vi "csb frames to pcap.vi"(0 "n_frames":i32, 1 "t_dev":dbl[](array[numeric]), 2 "id":u32[](array[numeric]), 3 "flags":u16[](array[numeric]), 4 "data_len":u8[](array[numeric]), 5 "data":u8[](array[numeric]), 6 "tai_minus_utc_s":i32, 7 "error in (no error)":errorcluster, 8 "options":i32, 9 "out":u8[](array[numeric])=array[4097 elements], 10 "out_cap":i32) -> (19 "out out":u8[](array[numeric]), 20 "n_packets":i32, 21 "n_skipped":i32, 22 "function return":i32, 27 "error out":errorcluster)   [LabVIEW 2021, in "CANsub_Codec.lvlib"]
doc: "int32_t csb_frames_to_pcap(int32_t n_frames, const double *t_dev, const uint32_t *id,\n const uint16_t *flags, const uint8_t *data_len, const uint8_t *data,\n int32_t tai_minus_utc_s, int32_t options,\n uint8_t *out, int32_t out_cap, int32_t *n_packets, int32_t *n_skipped);"
uses:
  CANsub_Codec.lvlib
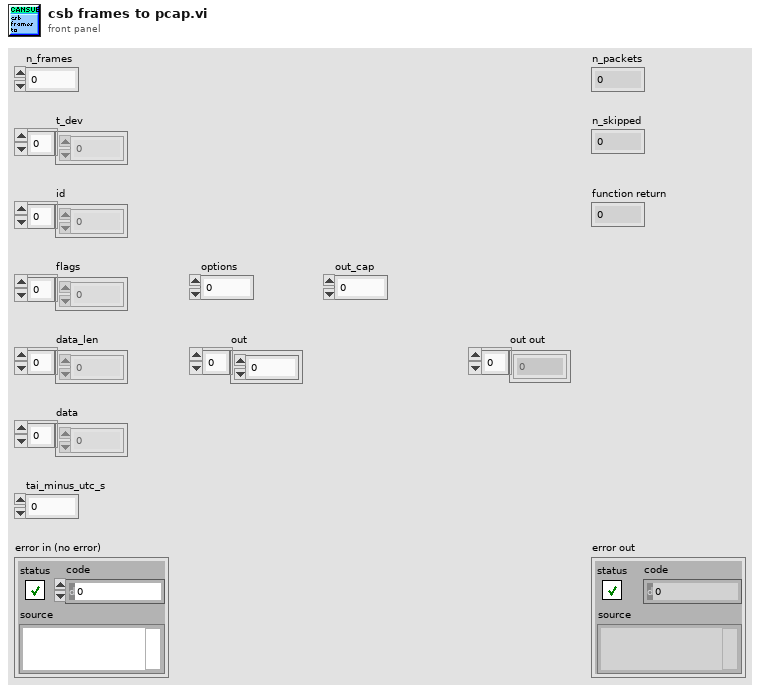
[diagram p1: front panel]
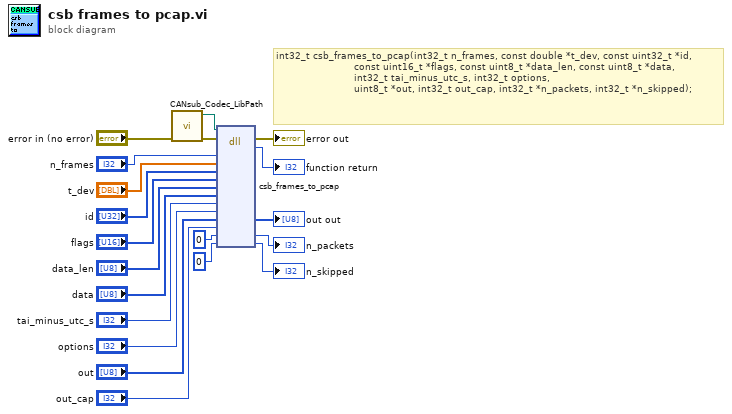
[diagram p0: block diagram]
diagram:
  # "int32_t csb_frames_to_pcap(int32_t n_frames, const double *t_dev, const uint32_t *id,\n                          const uint16_t *flags, const uint8_t *data_len, const uint8_t *data,\n                          int32_t tai_minus_utc_s, int32_t options,\n                          uint8_t *out, int32_t out_cap, int32_t *n_packets, int32_t *n_skipped);"
  n1 = call "CANsub_Codec_LibPath.vi"() -> ("Path"=w1:path)  [unwired: 11 in]
  n2 = dll-call lib="libcansub_codec.*" fn="csb_frames_to_pcap"(path in=w1, error in="error in (no error)", "n_frames"="n_frames", "t_dev"="t_dev", "id"="id", "flags"="flags", "data_len"="data_len", "data"="data", "tai_minus_utc_s"="tai_minus_utc_s", "options"="options", "out"="out", "out_cap"="out_cap", "n_packets"=0, "n_skipped"=0) -> (error out=→"error out":errorcluster, "return type"=→"function return":i32, "out"=→"out out":u8[], "n_packets"=→"n_packets":i32, "n_skipped"=→"n_skipped":i32)  [unwired: 10 in, 1 out]
